vi "SimulatorControlOscilloscope.vi"() -> ()   [LabVIEW 2014]
uses:
  SimulatorGlobalOscilloscope.vi
panel:
  out "Telemetry from LabviewOscilloscope":string
  out "Telecommand to LabviewOscilloscope":string
  in  "SEND":bool
  in  "Telecommand Packet":string
  # "SimulatorControlOscilloscpoe"
  # "Telecommands"
  # "Telemetry"
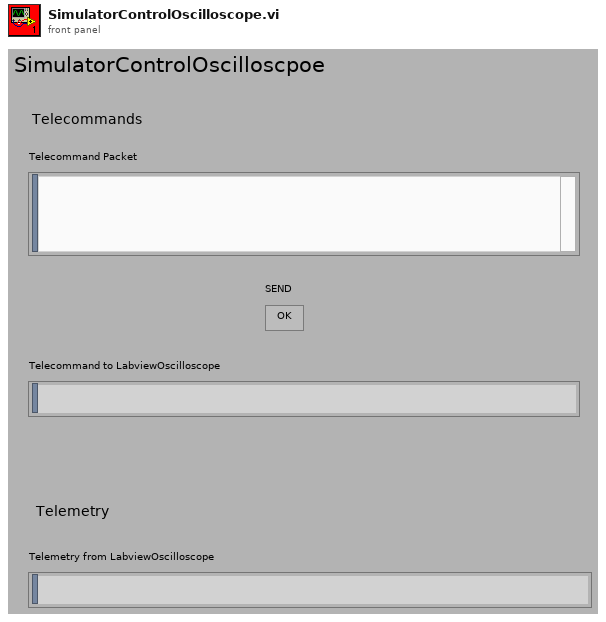
[diagram p1: front panel]
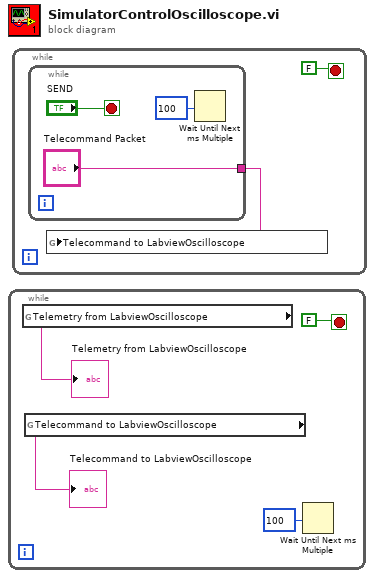
[diagram p0: block diagram]
diagram:
  n1 = while {
    stop <- FALSE stop-if-true
    n2 = global read "SimulatorGlobalOscilloscope.vi" "Telemetry from LabviewOscilloscope"() -> (→"Telemetry from LabviewOscilloscope":string)
    n3 = global read "SimulatorGlobalOscilloscope.vi" "Telecommand to LabviewOscilloscope"() -> (→"Telecommand to LabviewOscilloscope":string)
    n4 = Wait Until Next ms Multiple(millisecond multiple=100) -> ()  [unwired: 1 out]
  }
  n5 = while {
    stop <- FALSE stop-if-true
    n6 = while {
      tunnel: ["Telecommand Packet"] -> w6
      stop <- "SEND" stop-if-true
      n7 = Wait Until Next ms Multiple(millisecond multiple=100) -> ()  [unwired: 1 out]
    }
    n8 = global write "SimulatorGlobalOscilloscope.vi" "Telecommand to LabviewOscilloscope"(w6) -> ()
  }
